vi "Graphs.vi"(6 "Delete Values":bool=TRUE, 7 "Avg Thermal conductivity":dbl, 8 "error in (no error)":errorcluster, 9 "Time":u32, 10 "Data In":dbl[](array[numeric]), 11 "Test ID":string) -> (0 "error out":errorcluster, 1 "size(s)":i32, 2 "DATA":dbl[][](array[numeric]))   [LabVIEW 2026]
uses:
  <vilib>/Utility/file.llb/Write Delimited Spreadsheet (DBL).vi
  <vilib>/Utility/file.llb/Read Delimited Spreadsheet (DBL).vi
  <userlib>/_OpenG.lib/time/time.llb/openg_time.lvlib
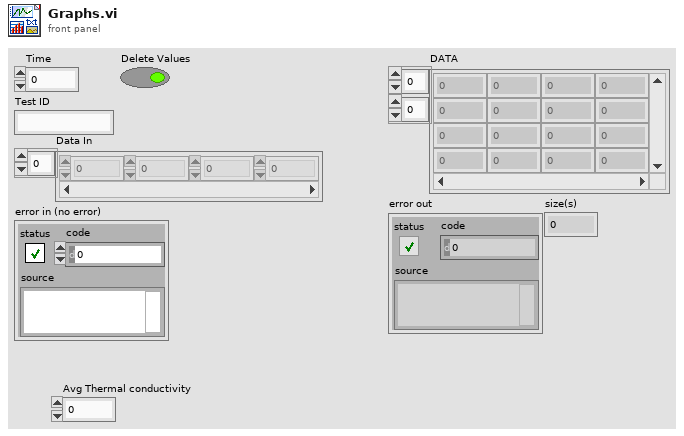
[diagram p1: front panel]
types:
  T1 = enum16{"open", "replace", "create", "open or create", "replace or create", "replace or create with confirmation"}
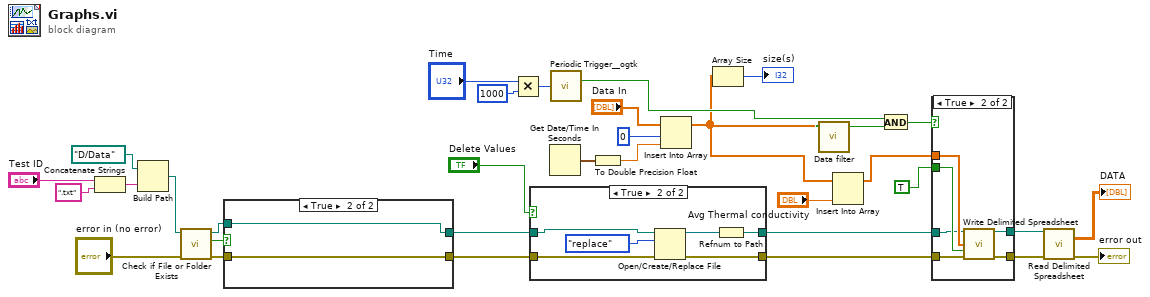
[diagram p0: block diagram]
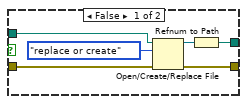
[diagram p4: hidden frame]
diagram:
  n1 = Concatenate Strings("Test ID", ".txt" ("string")) -> (w32:string)
  n2 = Build Path(base path=path "D:/Data", name or relative path=w32) -> (appended path=w22:path)
  n3 = call <vilib>:"Check if File or Folder Exists.vi"("error in (no error)"="error in (no error)", "path"=w22) -> ("error out"=w21:errorcluster, "file or folder exists?"=w20:bool, "dup path"=w19:path)  [unwired: 7 in]
  n4 = case shown="True" w20 {
    tunnel: w21 -> [w39 w41]
    tunnel: [w38 w41] -> w9
    tunnel: w19 -> [w37 w40]
    tunnel: [w35 w40] -> w18
    frame False {
      n5 = Open/Create/Replace File(file path (use dialog)=w37, error in=w39, operation (0:open)=T1."replace or create") -> (refnum out=w36:refnum<file>, error out=w38:errorcluster)  [unwired: 3 in, 1 out]
      n6 = Refnum to Path(1:w36) -> (0:w35:path)
    }
    frame True {
    }
  }
  n7 = Multiply(x="Time", y=u32 1000) -> (x*y=w14:u32)
  n8 = case shown="True" "Delete Values" {
    tunnel: w18 -> [w43 w49]
    tunnel: [w43 w45] -> w10
    tunnel: w9 -> [w42 w47]
    tunnel: [w42 w46] -> w8
    frame False {
    }
    frame True {
      n9 = Open/Create/Replace File(file path (use dialog)=w49, error in=w47, operation (0:open)=T1."replace") -> (refnum out=w48:refnum<file>, error out=w46:errorcluster)  [unwired: 3 in, 1 out]
      n10 = Refnum to Path(1:w48) -> (0:w45:path)
    }
  }
  n11 = Get Date/Time In Seconds() -> (seconds since 1Jan1904=w24:timestamp)
  n12 = call <userlib>:"Periodic Trigger__ogtk.vi"("time (ms)"=w14) -> ("Triggered"=w5:bool)  [unwired: 12 in, 2 out]
  n13 = To Double Precision Float(number=w24) -> (double precision float=w23:dbl)
  n14 = Insert Into Array "Insert Into Array"(array="Data In", index=0, new element=w23) -> (w3:dbl[])
  n15 = Array Size(array=w3) -> (size(s)=→"size(s)":i32)
  n16 = call "Data filter.vi"("Array"=w3) -> ("True"=w6:bool)  [unwired: 10 in]
  n17 = Insert Into Array(array=w3, new element="Avg Thermal conductivity") -> (w1:dbl[])  [unwired: 1 in]
  n18 = And(x=w5, y=w6) -> (x .and. y?=w4:bool)
  n19 = case shown="True" w4 {
    tunnel: [w51 w57] -> w29
    tunnel: [w50 w56] -> w28
    tunnel: TRUE ("append to file? (new file:F)") -> [_ w55]
    tunnel: w1 -> [_ w54]
    tunnel: w8 -> [w50 w53]
    tunnel: w10 -> [w51 w52]
    frame False {
    }
    frame True {
      n20 = call-poly <vilib>:"Write Delimited Spreadsheet.vi"("file path (dialog if empty)"=w52, "1D data"=w54, "append to file? (new file:F)"=w55, "error in (no error)"=w53) -> ("new file path (Not A Path if cancelled)"=w57:path, "error out"=w56:errorcluster)  [unwired: 10 in]
    }
  }
  n21 = call-poly <vilib>:"Read Delimited Spreadsheet.vi"("file path (dialog if empty)"=w29, "error in (no error)"=w28) -> ("all rows"=→"DATA":dbl[][], "error out"=→"error out":errorcluster)  [unwired: 8 in, 4 out]
